vi "Set Logger Enqueuer.vi"(8 "error in":errorcluster, 10 "Logger":refnum<class "Message Enqueuer.lvclass">, 11 "Hash Whitelist Handler in":refnum<class "Hash Whitelist Handler.lvclass">) -> (0 "error out":errorcluster, 3 "Hash Whitelist Handler out":refnum<class "Hash Whitelist Handler.lvclass">)   [LabVIEW 2026, in "Hash Whitelist Handler.lvclass"]
doc: "Set the logger enqueuer for a Logger Client."
uses:
  <vilib>/ActorFramework/Message Enqueuer/Message Enqueuer.lvclass
  Hash Whitelist Handler.lvclass
  Hash Whitelist Handler.lvclass/Hash Whitelist Handler.ctl
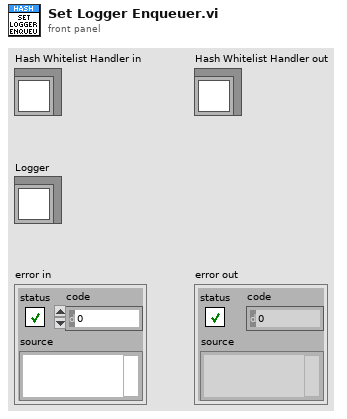
[diagram p1: front panel]
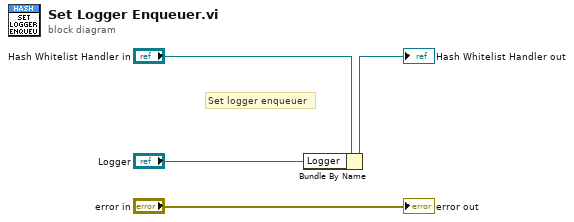
[diagram p0: block diagram]
diagram:
  # "Set logger enqueuer"
  n1 = Bundle By Name(cluster="Hash Whitelist Handler in", "Logger"="Logger") -> (→"Hash Whitelist Handler out":refnum<class "Hash Whitelist Handler.lvclass">)
  "error out" <- "error in"
